vi "Post-Install Custom Action.vi"(10 "Variant":variant) -> (0 "error out":errorcluster)   [LabVIEW 2020]
uses:
  <vilib>/Utility/config.llb/Write Key (Boolean).vi
  <vilib>/Utility/config.llb/Read Key (String).vi
  <vilib>/Utility/config.llb/Write Key (String).vi
  <vilib>/Utility/config.llb/NI_LVConfig.lvlib
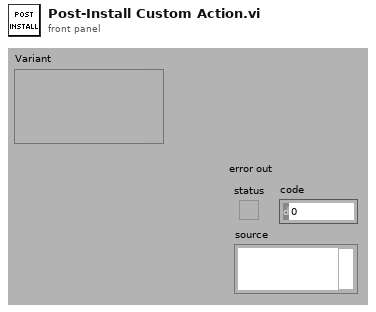
[diagram p1: front panel]
types:
  T1 = typedef "NI_LVConfig.lvlib/Config Data RefNum.ctl" = refnum<k1>
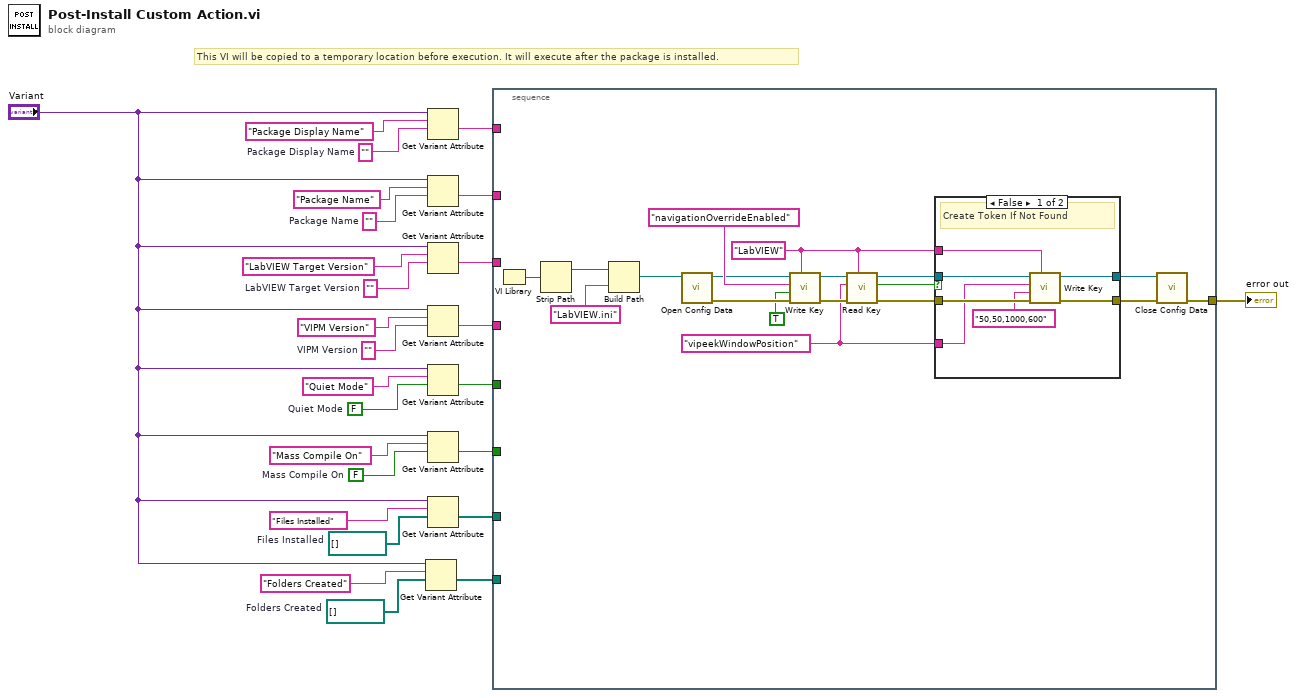
[diagram p0: block diagram]
diagram:
  w2 = path[] []  # Folders Created
  w3 = path[] []  # Files Installed
  w9 = FALSE  # Mass Compile On
  w10 = ""  # Package Display Name
  w17 = FALSE  # Quiet Mode
  w20 = ""  # VIPM Version
  w22 = ""  # LabVIEW Target Version
  w24 = ""  # Package Name
  # "This VI will be copied to a temporary location before execution. It will execute after the package is installed."
  n1 = Get Variant Attribute(Variant="Variant", name="Folders Created", default value (empty Variant)=w2) -> (value=w7:path[])  [unwired: 1 in, 3 out]
  n2 = Get Variant Attribute(Variant="Variant", name="Package Display Name", default value (empty Variant)=w10) -> (value=w16:string)  [unwired: 1 in, 3 out]
  n3 = Get Variant Attribute(Variant="Variant", name="Package Name", default value (empty Variant)=w24) -> (value=w15:string)  [unwired: 1 in, 3 out]
  n4 = Get Variant Attribute(Variant="Variant", name="LabVIEW Target Version", default value (empty Variant)=w22) -> (value=w14:string)  [unwired: 1 in, 3 out]
  n5 = Get Variant Attribute(Variant="Variant", name="VIPM Version", default value (empty Variant)=w20) -> (value=w13:string)  [unwired: 1 in, 3 out]
  n6 = Get Variant Attribute(Variant="Variant", name="Quiet Mode", default value (empty Variant)=w17) -> (value=w12:bool)  [unwired: 1 in, 3 out]
  n7 = Get Variant Attribute(Variant="Variant", name="Mass Compile On", default value (empty Variant)=w9) -> (value=w11:bool)  [unwired: 1 in, 3 out]
  n8 = Get Variant Attribute(Variant="Variant", name="Files Installed", default value (empty Variant)=w3) -> (value=w6:path[])  [unwired: 1 in, 3 out]
  n9 = stacked-sequence {
    tunnel: w16 -> [_]
    tunnel: w15 -> [_]
    tunnel: w14 -> [_]
    tunnel: w13 -> [_]
    tunnel: w12 -> [_]
    tunnel: w11 -> [_]
    tunnel: w6 -> [_]
    tunnel: w7 -> [_]
    tunnel: [w37] -> w1
    frame #0 {
      w28 = "vipeekWindowPosition" ("section")
      w27 = "LabVIEW" ("section")
      n10 = VI Library() -> (path=w44:path)
      n11 = Strip Path(path=w44) -> (stripped path=w43:path)  [unwired: 1 out]
      n12 = Build Path(base path=w43, name or relative path="LabVIEW.ini") -> (appended path=w36:path)
      n13 = call <vilib>:"Open Config Data.vi"("configuration file path"=w36) -> ("error out"=w41:errorcluster, "refnum"=w39:T1)  [unwired: 8 in, 1 out]
      n14 = call-poly <vilib>:"Write Key.vi"("section"=w27, "error in (no error)"=w41, "value"=TRUE, "key"="navigationOverrideEnabled" ("section"), "refnum"=w39) -> ("error out"=w34:errorcluster, "refnum out"=w35:T1)  [unwired: 4 in, 1 out]
      n15 = call-poly <vilib>:"Read Key.vi"("section"=w27, "error in (no error)"=w34, "key"=w28, "refnum"=w35) -> ("error out"=w31:errorcluster, "found?"=w33:bool, "refnum out"=w32:T1)  [unwired: 4 in, 1 out]
      n16 = case shown="False" w33 {
        tunnel: w32 -> [w49 w52]
        tunnel: w31 -> [w51 w53]
        tunnel: [w46 w53] -> w30
        tunnel: [w47 w52] -> w29
        tunnel: w28 -> [w50 _]
        tunnel: w27 -> [w48 _]
        frame False {
          # "Create Token If Not Found"
          n17 = call-poly <vilib>:"Write Key.vi"("section"=w48, "error in (no error)"=w51, "value"="50,50,1000,600" ("section"), "key"=w50, "refnum"=w49) -> ("error out"=w46:errorcluster, "refnum out"=w47:T1)  [unwired: 4 in, 1 out]
        }
        frame True {
          # "Don't Overwrite Token If Found"
        }
      }
      n18 = call <vilib>:"Close Config Data.vi"("error in (no error)"=w30, "refnum"=w29) -> ("error out"=w37:errorcluster)  [unwired: 8 in, 1 out]
    }
  }
  "error out" <- w1
